vi "VIH Dialog - About.vi"(8 "error in":errorcluster) -> (0 "error out":errorcluster)   [LabVIEW 2014]
doc: "::: VI Helpeks :::\nCopyright (c) 2000-2026 Konstantin Shifershteyn. All rights reserved."
uses:
  <vilib>/Platform/browser.llb/Open URL in Default Browser (string).vi
  <vilib>/Utility/cursorutil.llb/Set Cursor (Icon Pict).vi
panel:
  out "LV Version":string="."
  out "version":string="version 1.0.0"
  in  "%Home Page":bool
  in  "%URL":bool
  in  "cancel":bool
  out "date":string="22-08-2012"
  out "copyright":string="Copyright (c) 2012-2026, Konstantin Shifershteyn"
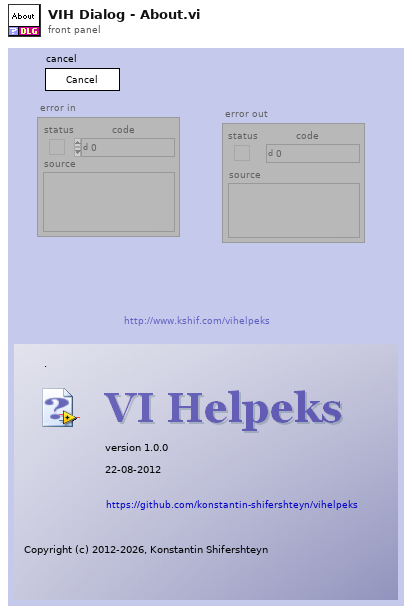
[diagram p1: front panel]
types:
  T1 = cluster{"Product Name":string, "Short Name":string, "Product Version":string, "Release Timestamp":string, "Developer":string, "Copyright":string}
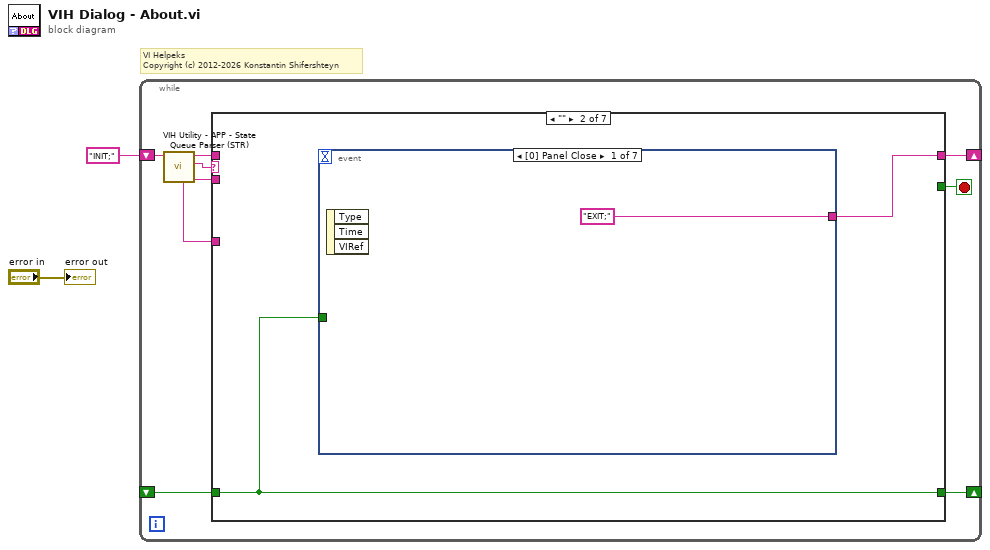
[diagram p0: block diagram]
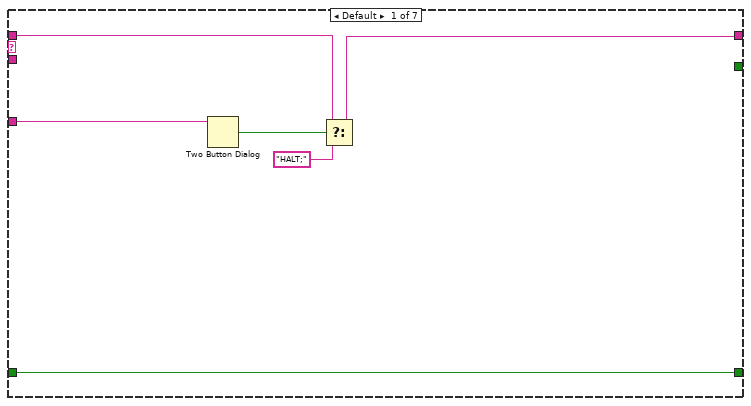
[diagram p2: hidden frame]
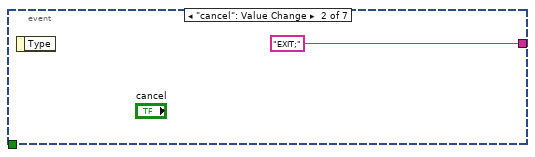
[diagram p3: hidden frame]
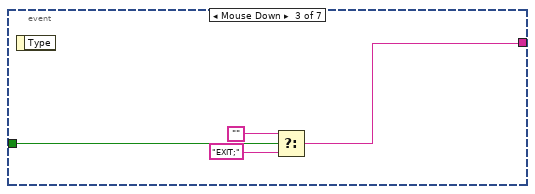
[diagram p4: hidden frame]
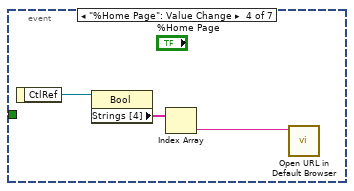
[diagram p5: hidden frame]
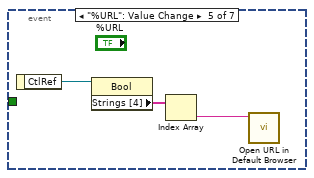
[diagram p6: hidden frame]
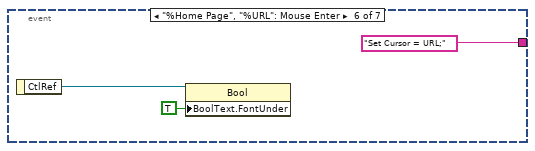
[diagram p7: hidden frame]
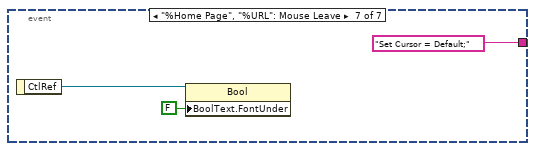
[diagram p8: hidden frame]
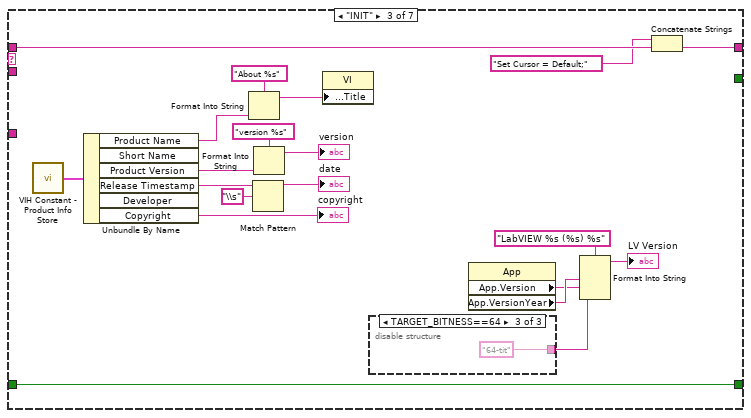
[diagram p9: hidden frame]
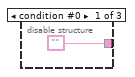
[diagram p10: hidden frame]
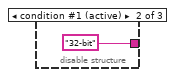
[diagram p11: hidden frame]
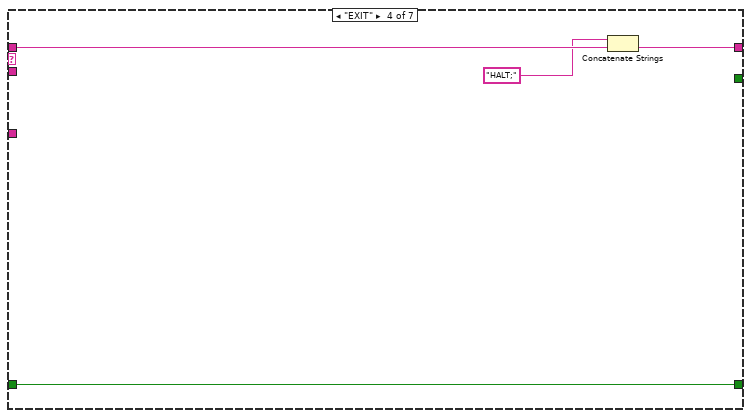
[diagram p12: hidden frame]
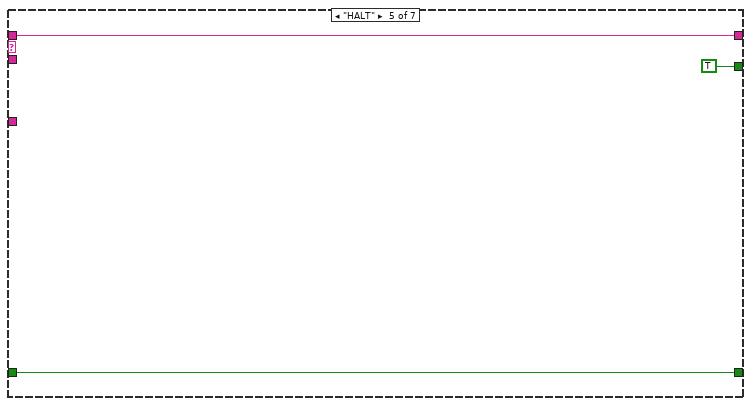
[diagram p13: hidden frame]
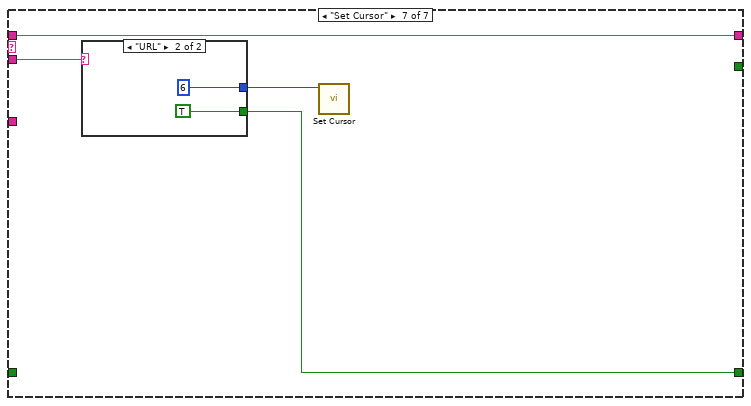
[diagram p15: hidden frame]
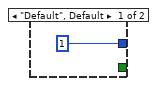
[diagram p16: hidden frame]
diagram:
  # "VI Helpeks\nCopyright (c) 2012-2026 Konstantin Shifershteyn"
  n1 = while {
    shift-right: [w7] -> _
    shift-left: "INIT;" -> [w11]
    shift-right: [w4] -> _
    shift-left: _ -> [w3]
    stop <- w6 stop-if-true
    n2 = call "VIH Utility - APP - State Queue Parser (STR).vi"("input queue"=w11) -> ("state parameters"=w5:string, "state"=w10:string, "remained queue"=w8:string, "complete state specifier"=w9:string)  [unwired: 5 in]
    n3 = case shown="\"\"" w10 {
      tunnel: w9 -> [w17 _ _ _ _ _ _]
      tunnel: w8 -> [w15 _ w49 w64 w67 w69 w73]
      tunnel: [w14 w19 w45 w63 w67 w69 w73] -> w7
      tunnel: [_ _ _ _ TRUE _ _] -> w6
      tunnel: w5 -> [_ _ _ _ _ _ w72]
      tunnel: [w12 w18 w43 w61 w65 w68 w70] -> w4
      tunnel: w3 -> [w12 w18 w43 w61 w65 w68 _]
      frame Default {
        n4 = Two Button Dialog(message=w17) -> (T button?=w16:bool)  [unwired: 2 in]
        n5 = Select(t=w15, s=w16, f="HALT;") -> (s? t:f=w14:string)
      }
      frame "" {
        n6 = event shown="[0] Panel Close" {
          selector: _ -> [_ _ _ _ _ _ _]
          dyn-events: _ -> [_ _ _ _ _ _ _]
          timeout: _ -> [_ _ _ _ _ _ _]
          tunnel: ["EXIT;" "EXIT;" w22 _ _ "Set Cursor = URL;" ("string") "Set Cursor = Default;" ("string")] -> w19
          tunnel: w18 -> [_ _ w25 _ _ _ _]
          event Panel Close {
            n7 = event-data() -> ()  [unwired: 1 in, 3 out]
          }
          event "cancel": Value Change {
            n8 = event-data() -> ()  [unwired: 1 in, 1 out]
          }
          event Mouse Down {
            n9 = event-data() -> ()  [unwired: 1 in, 1 out]
            n10 = Select(t="", s=w25, f="EXIT;") -> (s? t:f=w22:string)
          }
          event "%Home Page": Value Change {
            n11 = event-data() -> ("CtlRef"=w26:refnum<vi>)  [unwired: 1 in]
            n12 = property on="Property Node" class="Bool"(reference=w26) -> ("Strings [4]"=w28:string[])  [unwired: 1 in, 2 out]
            n13 = Index Array(array=w28) -> (element=w27:string)  [unwired: 1 in]
            n14 = call-poly <vilib>:"Open URL in Default Browser.vi"("URL"=w27) -> ()  [unwired: 5 in, 2 out]
          }
          event "%URL": Value Change {
            n15 = event-data() -> ("CtlRef"=w30:refnum<vi>)  [unwired: 1 in]
            n16 = property on="Property Node" class="Bool"(reference=w30) -> ("Strings [4]"=w31:string[])  [unwired: 1 in, 2 out]
            n17 = Index Array(array=w31) -> (element=w29:string)  [unwired: 1 in]
            n18 = call-poly <vilib>:"Open URL in Default Browser.vi"("URL"=w29) -> ()  [unwired: 5 in, 2 out]
          }
          event "%Home Page", "%URL": Mouse Enter {
            n19 = event-data() -> ("CtlRef"=w34:refnum<vi>)  [unwired: 1 in]
            n20 = property on="Property Node" class="Bool"(reference=w34, "BoolText.FontUnder"=TRUE ("Boolean Text.Font:Underline")) -> ()  [unwired: 1 in, 2 out]
          }
          event "%Home Page", "%URL": Mouse Leave {
            n21 = event-data() -> ("CtlRef"=w37:refnum<vi>)  [unwired: 1 in]
            n22 = property on="Property Node" class="Bool"(reference=w37, "BoolText.FontUnder"=FALSE ("Boolean Text.Font:Underline")) -> ()  [unwired: 1 in, 2 out]
          }
        }
      }
      frame "INIT" {
        n23 = call "VIH Constant - Product Info Store.vi"() -> ("Product Info"=w57:T1)
        n24 = Unbundle By Name(w57) -> ("Product Name"=w46:string, "Product Version"=w52:string, "Release Timestamp"=w56:string, "Copyright"=→"copyright":string)  [unwired: 2 out]
        n25 = Format Into String(format string="About %s", w46) -> (resulting string=w47:string)  [unwired: 2 in, 1 out]
        n26 = Match Pattern(string=w56, regular expression="\\s") -> (before substring=→"date":string)  [unwired: 1 in, 3 out]
        n27 = Format Into String(format string="version %s", w52) -> (resulting string=→"version":string)  [unwired: 2 in, 1 out]
        n28 = property class="VI"("Front Panel.Title"=w47) -> ()  [unwired: 2 in, 2 out]
        n29 = disable-structure shown="TARGET_BITNESS==64" {
          disable-tunnel: ["" "32-bit" "64-tit"] -> w38
          frame condition #0 {
          }
          frame condition #1 (active) {
          }
          frame condition #2 {
          }
        }
        n30 = property class="App"() -> ("App.Version"=w40:string, "App.VersionYear"=w41:string)  [unwired: 2 in, 2 out]
        n31 = Format Into String(format string="LabVIEW %s (%s) %s" ("string"), w41, w40, w38) -> (resulting string=→"LV Version":string)  [unwired: 2 in, 1 out]
        n32 = Concatenate Strings("Set Cursor = Default;" ("string"), w49) -> (w45:string)
      }
      frame "EXIT" {
        n33 = Concatenate Strings("HALT;", w64) -> (w63:string)
      }
      frame "HALT" {
      }
      frame "------------------------------ 1" {
      }
      frame "Set Cursor" {
        n34 = case shown="\"URL\"" w72 {
          tunnel: [u16 1 ("icon") u16 6 ("icon")] -> w71
          tunnel: [_ TRUE] -> w70
          frame "Default", Default {
          }
          frame "URL" {
          }
        }
        n35 = call-poly <vilib>:"Set Cursor.vi"("icon"=w71) -> ()  [unwired: 9 in, 2 out]
      }
    }
  }
  "error out" <- "error in"
